vi "Async.Engine.Initialize.vi"(7 "Error Log Settings":T1, 8 "error in (no error)":errorcluster, 10 "Processes":cluster{"VI":refnum<vi>, "Parameters":variant}[](array[cluster]), 11 "Custom Device Ref":T2 format="%.0x") -> (0 "error out":errorcluster, 3 "Async":refnum<class "VS Inline Async API.lvclass">)   [LabVIEW 2015, in "VS Inline Async API.lvlib" / "VS Inline Async API.lvclass"]
uses:
  VS Inline Async API.lvclass
  <vilib>/NI Veristand/Custom Device API/Custom Device Item Ref.ctl
  Types/Error Handling Settings.ctl
  VS Inline Async API.lvclass/VS Inline Async API.ctl
  Error Handling Process/SubVIs/Error.GetError.vi
  <vilib>/Utility/error.llb/Error Cluster From Error Code.vi
  VS Inline Async API.lvlib
  _Data Access Engine/Data Access Engine/Data Access Engine.lvclass
  <vilib>/NI Veristand/Custom Device API/Custom Device API.lvlib
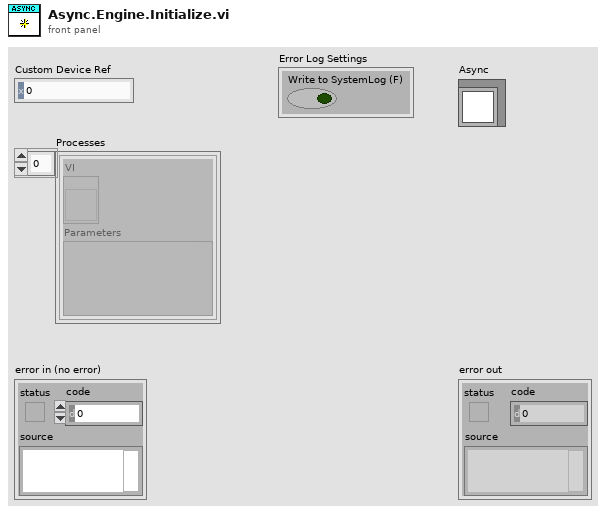
[diagram p1: front panel]
types:
  T1 = typedef "VS Inline Async API.lvlib/VS Inline Async API.lvclass/Error Handling Settings.ctl" = cluster{"Write to SystemLog (F)":bool}
  T2 = typedef "Custom Device API.lvlib/Custom Device Item Ref.ctl" = u64
  T3 = typedef "Custom Device API.lvlib/Custom Device Item Info.ctl" = cluster{"Name":string, "Is Channel":bool, "GUID":string, "Is Waveform":bool}
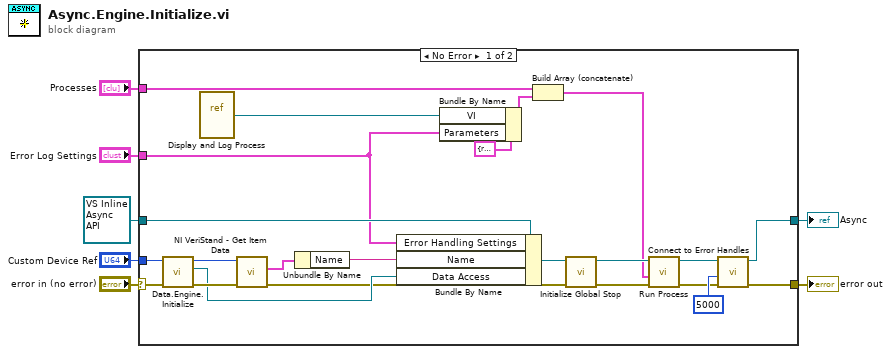
[diagram p0: block diagram]
diagram:
  n1 = case shown="No Error" "error in (no error)" {
    selector: "error in (no error)" -> [w17 w32]
    tunnel: [w26 w32] -> w6
    tunnel: [w24 w31] -> w4
    tunnel: refnum<class "VS Inline Async API.lvclass"> refnum ("Async in") -> [w29 w31]
    tunnel: "Processes" -> [w28 _]
    tunnel: "Custom Device Ref" -> [w16 _]
    tunnel: "Error Log Settings" -> [w8 _]
    frame No Error {
      n2 = call "Data.Engine.Initialize.vi"("error in"=w17, "Custom Device Ref"=w16) -> ("error out"=w15:errorcluster, "Data Access Engine"=w11:refnum<class "Data Access Engine.lvclass">, "Custom Device Ref"=w14:T2)  [unwired: 7 in]
      n3 = vi-ref "Display and Log Process.vi"() -> (w22:refnum<vi>)
      n4 = call <vilib>:"NI VeriStand - Get Item Data.vi"("error in (no error)"=w15, "Item Ref in"=w14) -> ("error out"=w10:errorcluster, "Item Info"=w13:T3)  [unwired: 6 in, 2 out]
      n5 = Unbundle By Name(w13) -> ("Name"=w12:string)
      n6 = Bundle By Name(cluster=w29, "Error Handling Settings"=w8, "Name"=w12, "Data Access"=w11) -> (w9:refnum<class "VS Inline Async API.lvclass">)
      n7 = Bundle By Name(cluster=cluster{"VI":refnum<vi>, "Parameters":variant} {"VI"=refnum, "Parameters"=variant} ("Process"), "VI"=w22, "Parameters"=w8) -> (w21:cluster{"VI":refnum<vi>, "Parameters":variant})
      n8 = Build Array (concatenate)(w28, w21) -> (w18:cluster{"VI":refnum<vi>, "Parameters":variant}[])
      n9 = call "Initialize Global Stop.vi"("error in (no error)"=w10, "Async in"=w9) -> ("error out"=w20:errorcluster, "Async out"=w19:refnum<class "VS Inline Async API.lvclass">)  [unwired: 8 in]
      n10 = call "Run Process.vi"("error in (no error)"=w20, "Processes"=w18, "Async in"=w19) -> ("error out"=w27:errorcluster, "Async out"=w25:refnum<class "VS Inline Async API.lvclass">)  [unwired: 7 in]
      n11 = call "Connect to Error Handles.vi"("error in"=w27, "Timeout (ms)"=u16 5000, "Async in"=w25) -> ("error out"=w26:errorcluster, "Async out"=w24:refnum<class "VS Inline Async API.lvclass">)  [unwired: 7 in]
    }
    frame Error {
    }
  }
  "error out" <- w6
  "Async" <- w4
